vi "example test.vi"() -> ()   [LabVIEW 2013, in "Profibus Module tests.lvlib"]
uses:
  Profibus Module tests.lvlib
  <vilib>/Utility/RT CPU Load.ctl
  configuration/Profibus Module configuration.lvclass
  execution/Profibus Module runtime.lvclass
  <vilib>/NI/Tag Bus/tag/Data Type.ctl
  <vilib>/NI/Tag Bus Module Framework/channel/channel classification.ctl
  channel/Profibus channel.lvclass
  <vilib>/userdefined/High Color/nirio_resource_hc.ctl
  <vilib>/NI/Tag Bus Module Framework/FPGA manager/methods.ctl
  <vilib>/Platform/TimedLoop/XDataNode/timing_clust.ctl
  <vilib>/Platform/TimedLoop/XDataNode/nitl_modes.ctl
  <vilib>/Platform/TimedLoop/XDataNode/wakeup.ctl
  configuration/endianness setting.ctl
  configuration/slave diagnostic configuration.ctl
  <vilib>/NI/Tag Bus Module Framework/channel/TBM channel.lvclass
  configuration/error throw specification.ctl
  <vilib>/NI/Tag Bus Module Framework/channel/TBM channel.lvclass/TBM channel.ctl
  channel/Profibus channel.lvclass/Profibus channel.ctl
  <vilib>/NI/Tag Bus/tag/tag descriptor.lvclass/tag descriptor.ctl
  configuration/Profibus Module configuration.lvclass/Profibus Module configuration.ctl
  <vilib>/NI/Tag Bus/dictionary/data dictionary.lvclass/data dictionary.ctl
  <vilib>/NI/Tag Bus/dictionary/lookup polymorphs/locate Array of U8.vi
  <vilib>/NI/Tag Bus/table/data polymorphs/write one/write U16.vi
  <vilib>/NI/Tag Bus/table/data polymorphs/write one/write Array of U8.vi
  <vilib>/NI/Tag Bus/table/data polymorphs/read one/read Array of U8.vi
  <vilib>/NI/Tag Bus Module Framework/channel/Write channel classification.vi
  channel/Write slave.vi
  channel/Write byte.vi
  channel/Write bit.vi
  <vilib>/NI/Tag Bus/tag/write data type.vi
  <vilib>/NI/Tag Bus/tag/write tag name.vi
  configuration/Write byte orders.vi
  configuration/Write slave diagnostics.vi
  <vilib>/NI/Tag Bus/dictionary/search/find data index.vi
  <vilib>/NI/Tag Bus/dictionary/search/search string list.vi
  <vilib>/FPGAPlugInAG/cRIO-9074/niLvFpga_Open_cRIO-9074.vi
  <vilib>/rvi/interface/common/dynamic/niFpgaDynamicAddResources.vi
  <vilib>/FPGAPlugInAG/Dynamic/niLvFpga_Reset_Dynamic.vi
  <vilib>/FPGAPlugInAG/Dynamic/niLvFpga_Run_Dynamic.vi
  <vilib>/NI/Tag Bus/dictionary/tag not found.vi
  <vilib>/rvi/interface/common/niFpgaWaitOnOcc.vi
  <vilib>/Utility/error.llb/Error Cluster From Error Code.vi
  <vilib>/rvi/errors/niLvFpgaAdjustHostInterfaceError.vi
  <vilib>/FPGAPlugInAG/Dynamic/niLvFpga_Close_Dynamic.vi
  <vilib>/platform/TimedLoop/XDataNode/XDataNode.xnode
  <vilib>/rvi/interface/nirviOpenFPGA/nirviOpenFPGA.xnode
  FPGA Bitfiles/ProfibusModule_FPGA9074_FPGAMain_bIHCZjrjays.lvbitx
  execution/FPGA Main.vi
  <vilib>/rvi/interface/nirviMethod/nirviMethod.xnode
  <vilib>/rvi/interface/nirviCloseFPGA/nirviCloseFPGA.xnode
  <vilib>/NI/Tag Bus/dictionary/data dictionary.lvclass
  <vilib>/NI/Tag Bus/table/data table.lvlib
  <vilib>/NI/Tag Bus/tag/tag descriptor.lvclass
  <vilib>/NI/Configuration Framework/serializable configuration/NISE_CEF_serializable configuration.lvclass
  <vilib>/NI/Tag Bus Module Framework/FPGA manager/FPGA manager.lvlib
  <vilib>/NI_Real-Time Target Support.lvlib
  <vilib>/Platform/TimedLoop/XDataNode/XDNodeRunTimeDep.lvlib
  <vilib>/FPGAPlugInAG/Dynamic/niLvFpga_ReadFifo_Dynamic.vi
  <vilib>/rvi/errors/niLvFpgaMergeErrorWithErrorCode.vi
  <vilib>/ptbypt/NI_PtbyPt.lvlib
  <vilib>/NI/Tag Bus/dictionary/lookup polymorphs/locate U16.vi
panel:
  out "class name":string
  out "configuration out":refnum<class "Profibus Module configuration.lvclass">
  out "diag":u8[](array[numeric])
  out "value":u8[](array[numeric])
  in  "value 2":u16
  out "*(type *) &x 2":u64
  out "rio init error":errorcluster
  out "in mean":dbl
  out "out mean":dbl
  out "out":dbl
  out "in":dbl
  out "Elements Remaining":u32
  in  "millisecond multiple":u32=100
  out "CPU loads":T1[](array[typedef]) {"ISR (%)" format="%#.2f"; "Idle (%)" format="%#.2f"; "Background (%)" format="%#.2f"; "Normal (%)" format="%#.2f"; "Above Normal (%)" format="%#.2f"; "High (%)" format="%#.2g"; "Timed Structures (%)" format="%#.2g"; "Time Critical (%)" format="%#.2g"; "Total (%)" format="%#.2g"}
  in  "stop cpu":bool
  out "*(type *) &x":u64
  out "error out":errorcluster
  in  "stop":bool
  out "final error":errorcluster
  out "output error":errorcluster
  out "input error":errorcluster
  out "output lookup error":errorcluster
  out "input lookup error":errorcluster
  out "init error":errorcluster
  out "correct execution settings":bool
  out "serialization problem":errorcluster
  out "invalid configuration":errorcluster
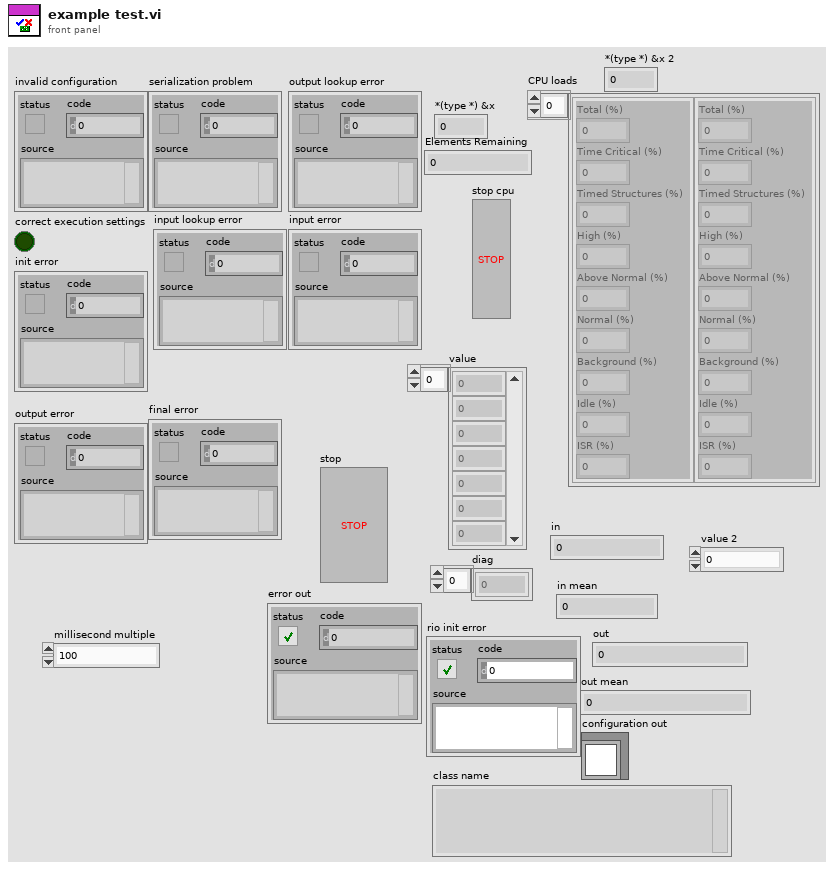
[diagram p1: front panel]
types:
  T1 = typedef "NI_Real-Time Target Support.lvlib/RT CPU Load.ctl" = cluster{"Total (%)":dbl, "Time Critical (%)":dbl, "Timed Structures (%)":dbl, "High (%)":dbl, "Above Normal (%)":dbl, "Normal (%)":dbl, "Background (%)":dbl, "Idle (%)":dbl, "ISR (%)":dbl}
  T2 = typedef "TBM channel.lvclass/channel classification.ctl" = enum16{"input data", "output data", "processing parameter", "processing result"}
  T3 = typedef "tag bus.lvlib/tag descriptor.lvclass/Data Type.ctl" = enum16{"Double", "Single", "I64", "I32", "I16", "I8", "U64", "U32", "U16", "U8", "Boolean", "String", "Array of Double", "Array of Single", "Array of I64", "Array of I32", "Array of I16", "Array of I8", "Array of U64", "Array of U32", "Array of U16", "Array of U8", "Array of Boolean", "Array of String"}
  T4 = typedef "Profibus Module configuration.lvclass/slave diagnostic configuration.ctl" = cluster{"slave":i8, "report":bool, "channel":refnum<class "TBM channel.lvclass">, "error specs":T5[]}
  T5 = typedef "Profibus Module configuration.lvclass/error throw specification.ctl" = cluster{"byte":i32, "bit":i32, "inverted?":bool, "error":i32}
  T6 = typedef "Profibus Module configuration.lvclass/endianness setting.ctl" = cluster{"slave":i8, "big endian":bool}
  T7 = typedef "nirio_resource_hc.ctl" = tag
  T8 = typedef "FPGA manager.lvlib/methods.ctl" = enum16{"initialize bitfile", "cache bitfile", "locate bitfile", "close bitfile", "clear manager"}
  T9 = typedef "TBM channel.lvclass/data tables.ctl" = cluster{"input data":T10, "processing parameter":T10, "processing result":T10, "output data":T10}
  T10 = typedef "tag bus.lvlib/dictionary table pair.ctl" = cluster{"data dictionary":refnum<class "data dictionary.lvclass">, "data table":T11}
  T11 = typedef "tag bus.lvlib/data table.lvlib/data table.ctl" = cluster{"Double":dbl[], "Single":sgl[], "I64":i64[], "I32":i32[], "I16":i16[], "I8":i8[], "U64":u64[], "U32":u32[], "U16":u16[], "U8":u8[], "Boolean":bool[], "String":string[], "Array of Double":cluster{"DBL Array":dbl[]}[], "Array of Single":cluster{"SGL Array":sgl[]}[], "Array of I64":cluster{"I64 Array":i64[]}[], "Array of I32":cluster{"I32 Array":i32[]}[], "Array of I16":cluster{"I16 Array":i16[]}[], "Array of I8":cluster{"I8 Array":i8[]}[], "Array of U64":cluster{"U64 Array":u64[]}[], "Array of U32":cluster{"U32 Array":u32[]}[], "Array of U16":cluster{"U16 Array":u16[]}[], "Array of U8":cluster{"U8 Array":u8[]}[], "Array of Boolean":cluster{"Boolean Array":bool[]}[], "Array of String":cluster{"String Array":string[]}[]}
  T12 = typedef "TBM module execution interface.lvclass/execution settings.ctl" = cluster{"reads inputs":bool, "processes data":bool, "writes outputs":bool}
  T13 = typedef "XDNodeRunTimeDep.lvlib/timing_clust.ctl" = cluster{"Expected End [f-1]":u64, "Actual End [f-1]":u64, "Finished Late? [f-1]":bool, "Expected End [i-1]":u64, "Actual End [i-1]":u64, "Finished Late? [i-1]":bool, "Expected Start [i]":u64, "Actual Start [i]":u64, "Expected Start [f]":u64, "Actual Start [f]":u64, "Source Name":string, "Structure Name":string, "Period":i64, "Deadline":i64, "Offset":i64, "Start":i64, "Priority":i32, "Timeout":i32, "Mode":T14, "Wakeup Reason":T15, "Error":errorcluster, "Source Type":string, "Secondary Source Type":string, "Global End Time":u64, "Global Start Time":u64, "Frame Duration":u64, "Iteration Duration":u64, "Assigned CPU":i32, "I/O Scan Engine Mode":u32}
  T14 = typedef "XDNodeRunTimeDep.lvlib/nitl_modes.ctl" = enum32{"No Change", "Process missed periods, maintain original phase", "Discard missed periods, maintain original phase", "Process missed periods, ignore original phase", "Discard missed periods, ignore original phase"}
  T15 = typedef "XDNodeRunTimeDep.lvlib/wakeup.ctl" = enum32{"Normal", "Aborted", "Asynchronous wakeup", "Timing source error", "Timed loop error", "Timeout"}
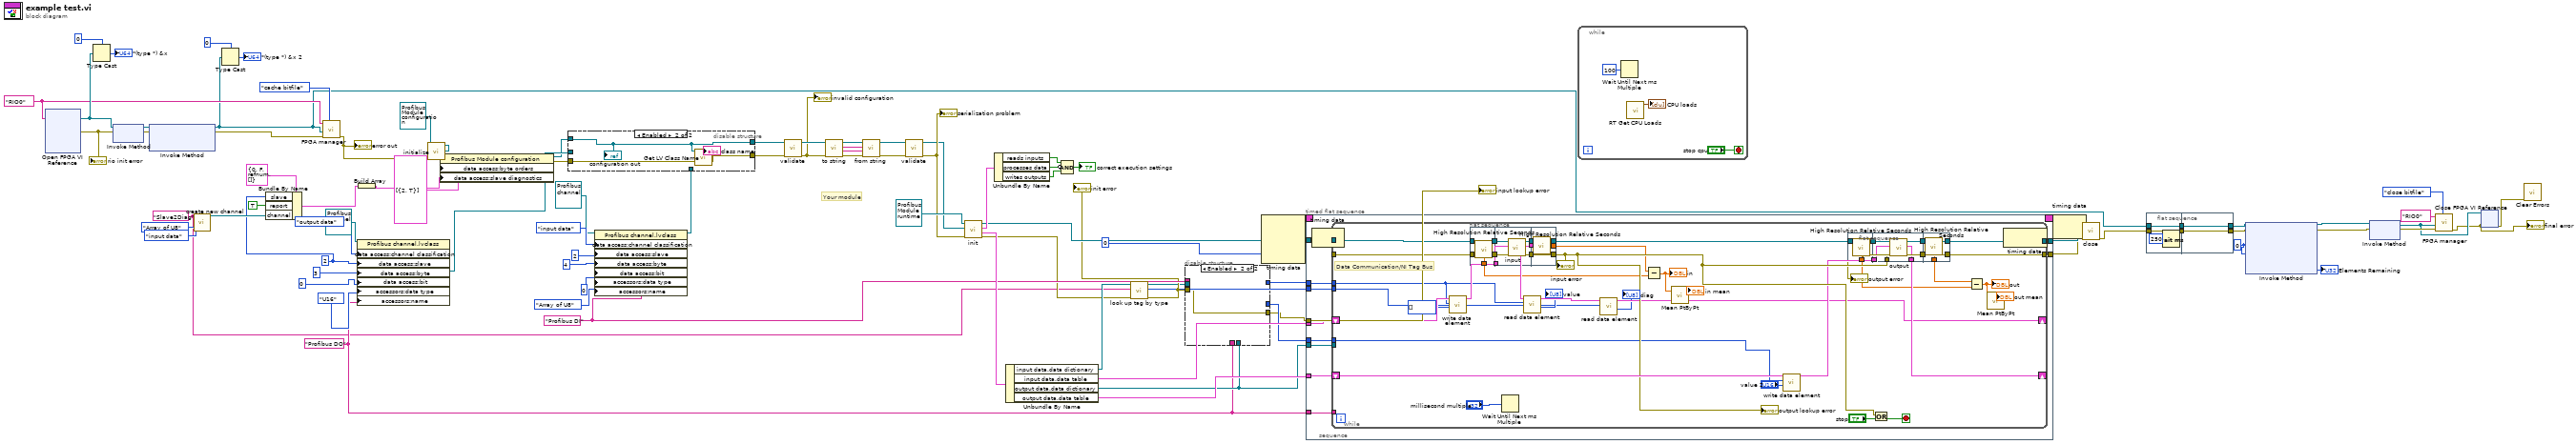
[diagram p0: block diagram]
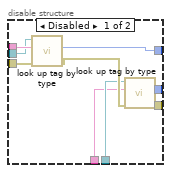
[diagram p2: hidden frame]
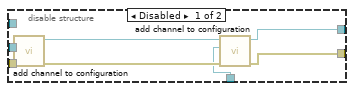
[diagram p3: hidden frame]
diagram:
  w4 = "Slave2Diag" ("channel name")
  w33 = u32 0 ("Number of Elements")
  w31 = T7 "RIO0" ("RIO resource")
  w54 = "Profibus DI" ("name")
  w11 = i8 2 ("slave")
  w18 = "Profibus DO" ("name")
  # "Your module"
  n1 = xnode "Open FPGA VI Reference"("resource name"=w31) -> ("FPGA VI Reference Out"=w45:refnum<k20>, "error out"=w53:errorcluster)  [unwired: 1 in]
  "rio init error" <- w53
  n2 = Type Cast(type=u64 0, x=w45) -> (*(type *) &x=→"*(type *) &x":u64)
  n3 = xnode "Invoke Method"("FPGA VI Reference In"=w45, "error in"=w53) -> ("FPGA VI Reference Out"=w51:refnum<k20>, "error out"=w52:errorcluster)
  n4 = xnode "Invoke Method"("FPGA VI Reference In"=w51, "error in"=w52) -> ("FPGA VI Reference Out"=w1:refnum<k20>, "error out"=w50:errorcluster)  [unwired: 1 in]
  n5 = call <vilib>:"create new channel.vi"("channel classification"=channel_classification."input data", "data type"=Data_Type."Array of U8", "channel name"=w4) -> ("channel"=w12:refnum<class "TBM channel.lvclass">)  [unwired: 8 in]
  n6 = Type Cast(type=u64 0, x=w1) -> (*(type *) &x=→"*(type *) &x 2":u64)
  n7 = Bundle By Name(cluster=T4 {"slave"=0, "report"=FALSE, "channel"=refnum, "error specs"=[]} ("diagnostics settings"), "slave"=w11, "report"=TRUE, "channel"=w12) -> (w15:T4)
  n8 = call <vilib>:"FPGA manager.vi"("action"=methods."cache bitfile", "error in"=w50, "bitfile to cache"=w1, "RIO resource"=w31) -> ("error out"=w48:errorcluster)  [unwired: 5 in, 2 out]
  "error out" <- w48
  n9 = property class="Profibus channel.lvclass"(reference=refnum<class "Profibus channel.lvclass"> refnum ("Profibus channel.lvclass"), "data access:channel classification"=channel_classification."output data" ("channel classification"), "data access:slave"=w11, "data access:byte"=3 ("DO byte"), "data access:bit"=0 ("DO bit"), "accessors:data type"=Data_Type."U16" ("data type"), "accessors:name"=w18) -> (reference out=w55:refnum<class "Profibus channel.lvclass">)  [unwired: 1 in, 1 out]
  n10 = Build Array(w15) -> (w14:T4[])
  n11 = call <vilib>:"initialize.vi"("error in"=w48, "configuration in"=refnum<class "Profibus Module configuration.lvclass"> refnum ("tag bus configurable plugin module configuration")) -> ("error out"=w68:errorcluster, "configuration out"=w23:refnum<class "Profibus Module configuration.lvclass">)  [unwired: 7 in, 1 out]
  n12 = property class="Profibus Module configuration"(reference=w23, error in=w68, "data access:byte orders"=T6[] [{"slave"=2, "big endian"=TRUE}] ("byte orders"), "data access:slave diagnostics"=w14) -> (reference out=w2:refnum<class "Profibus Module configuration.lvclass">, error out=w24:errorcluster)
  n13 = property class="Profibus channel.lvclass"(reference=refnum<class "Profibus channel.lvclass"> refnum ("Profibus channel.lvclass"), "data access:channel classification"=channel_classification."input data" ("channel classification"), "data access:slave"=i8 2 ("slave"), "data access:byte"=4 ("DI byte"), "data access:bit"=0 ("DI bit"), "accessors:data type"=Data_Type."Array of U8" ("data type"), "accessors:name"=w54) -> (reference out=w56:refnum<class "Profibus channel.lvclass">)  [unwired: 1 in, 1 out]
  n14 = disable-structure shown="Enabled" {
    disable-tunnel: [w101 w103] -> w71
    disable-tunnel: [w100 w104] -> w70
    disable-tunnel: w56 -> [w97 _]
    disable-tunnel: w55 -> [w96 _]
    disable-tunnel: w24 -> [w95 w104]
    disable-tunnel: w2 -> [_ w103]
    frame Disabled {
      n15 = call "add channel to configuration.vi"("error in"=w95, "TBM channel in"=w96) -> ("error out"=w98:errorcluster, "Profibus Module configuration out"=w99:refnum<class "Profibus Module configuration.lvclass">)  [unwired: 8 in]
      n16 = call "add channel to configuration.vi"("error in"=w98, "TBM channel in"=w97, "Profibus Module configuration in"=w99) -> ("error out"=w100:errorcluster, "Profibus Module configuration out"=w101:refnum<class "Profibus Module configuration.lvclass">)  [unwired: 7 in]
    }
    frame Enabled {
      n17 = call <vilib>:"Get LV Class Name.vi"("object"=w103) -> ("class name"=→"class name":string)  [unwired: 9 in, 1 out]
      "configuration out" <- w103
    }
  }
  n18 = call-dynamic "validate.vi"("error in"=w70, "Profibus Module configuration in"=w71) -> ("error out"=w93:errorcluster, "Profibus Module configuration out"=w94:refnum<class "Profibus Module configuration.lvclass">)  [unwired: 8 in]
  "invalid configuration" <- w93
  n19 = call-dynamic "to string.vi"("error in"=w93, "Profibus Module configuration in"=w94) -> ("error out"=w89:errorcluster, "data"=w90:string, "version"=w91:string, "Profibus Module configuration out"=w92:refnum<class "Profibus Module configuration.lvclass">)  [unwired: 6 in]
  n20 = call-dynamic "from string.vi"("error in"=w89, "data"=w90, "version"=w91, "Profibus Module configuration in"=w92) -> ("error out"=w87:errorcluster, "Profibus Module configuration out"=w88:refnum<class "Profibus Module configuration.lvclass">)  [unwired: 6 in]
  n21 = call-dynamic "validate.vi"("error in"=w87, "Profibus Module configuration in"=w88) -> ("error out"=w85:errorcluster, "Profibus Module configuration out"=w84:refnum<class "Profibus Module configuration.lvclass">)  [unwired: 8 in]
  "serialization problem" <- w85
  n22 = call-dynamic "init.vi"("error in"=w85, "TBM module configuration in"=w84, "Profibus Module runtime in"=refnum<class "Profibus Module runtime.lvclass"> refnum ("tag bus configurable plugin module")) -> ("error out"=w5:errorcluster, "data allocations"=w78:T9, "execution settings"=w83:T12, "Profibus Module runtime out"=w76:refnum<class "Profibus Module runtime.lvclass">)  [unwired: 5 in]
  n23 = Unbundle By Name(w83) -> ("reads inputs"=w80:bool, "processes data"=w82:bool, "writes outputs"=w81:bool)
  n24 = Unbundle By Name(w78) -> ("input data.data dictionary"=w7:refnum<class "data dictionary.lvclass">, "input data.data table"=w77:T11, "output data.data dictionary"=w20:refnum<class "data dictionary.lvclass">, "output data.data table"=w74:T11)
  n25 = Compound Arithmetic op=AND(w80, invert w82, w81) -> (→"correct execution settings":bool)
  n26 = call-poly <vilib>:"look up tag by type.vi"("error in"=w5, "name"=w4, "data dictionary in"=w7) -> ("error out"=w8:errorcluster, "index"=w3:i32, "data dictionary out"=w6:refnum<class "data dictionary.lvclass">)  [unwired: 6 in]
  "init error" <- w8
  n27 = disable-structure shown="Enabled" {
    disable-tunnel: [w113 _] -> w75
    disable-tunnel: w54 -> [w112 _]
    disable-tunnel: w20 -> [w110 _]
    disable-tunnel: [w109 _] -> w19
    disable-tunnel: w18 -> [w108 _]
    disable-tunnel: [w107 w114] -> w17
    disable-tunnel: w8 -> [w106 w114]
    disable-tunnel: w6 -> [w105 _]
    frame Disabled {
      n28 = call-poly <vilib>:"look up tag by type.vi"("error in"=w106, "name"=w112, "data dictionary in"=w105) -> ("error out"=w111:errorcluster, "index"=w113:i32)  [unwired: 6 in, 1 out]
      n29 = call-poly <vilib>:"look up tag by type.vi"("error in"=w111, "name"=w108, "data dictionary in"=w110) -> ("error out"=w107:errorcluster, "index"=w109:i32)  [unwired: 6 in, 1 out]
    }
    frame Enabled {
    }
  }
  "input lookup error" <- w17
  n30 = node-c288(0 ("Processor")) -> (w42:T13)  [unwired: 3 in]
  n31 = timed-sequence {
    timing: w42 -> [_]
    timing-out: [_] -> w41
    tunnel: w77 -> [w125]
    tunnel: w76 -> [w124]
    tunnel: w17 -> [w123]
    tunnel: w75 -> [w122]
    tunnel: w20 -> [w121]
    tunnel: w74 -> [w120]
    tunnel: [w119] -> w73
    tunnel: [w118] -> w72
    tunnel: w18 -> [w117]
    tunnel: w19 -> [w116]
    tunnel: w3 -> [w115]
    n32 = timed-flat-sequence {
      tunnel: w125 -> [w136]
      tunnel: w124 -> [w135]
      tunnel: w123 -> [w134]
      tunnel: w122 -> [w133]
      tunnel: w121 -> [w132]
      tunnel: w120 -> [w131]
      tunnel: [w130] -> w119
      tunnel: [w129] -> w118
      tunnel: w117 -> [w128]
      tunnel: w116 -> [w127]
      tunnel: w115 -> [w126]
      n33 = node-c288() -> ()  [unwired: 1 in, 1 out]
      n34 = while {
        tunnel: w135 -> [w175]
        tunnel: w134 -> [w174]
        tunnel: w133 -> [w171]
        tunnel: w132 -> [_]
        tunnel: [w166] -> w130
        tunnel: [w161] -> w129
        shift-right: [w165] -> _
        shift-left: w131 -> [w170]
        shift-right: [w139] -> _
        shift-left: w136 -> [w176]
        tunnel: w128 -> [_]
        tunnel: w127 -> [w143]
        tunnel: w126 -> [w138]
        stop <- w144 stop-if-true
        # "Data Communication/NI Tag Bus"
        n35 = call-poly <vilib>:"write data element.vi"("value"=u8[] [], "index"=w171, "data table in"=w176) -> ("data table out"=w173:T11)  [unwired: 8 in]
        n36 = flat-sequence {
          tunnel: w174 -> [w189]
          tunnel: w175 -> [w190]
          tunnel: [w190] -> w157
          tunnel: [w189] -> w156
          tunnel: [w188] -> w151
          tunnel: w173 -> [w194]
          tunnel: [w193] -> w160
          tunnel: [w192] -> w159
          tunnel: [w191] -> w158
          tunnel: w157 -> [w196]
          tunnel: w156 -> [w195]
          tunnel: [w198] -> w168
          tunnel: [w199] -> w169
          tunnel: [w200] -> w172
          tunnel: w160 -> [w200]
          tunnel: w159 -> [w199]
          tunnel: w158 -> [w198]
          tunnel: [w197] -> w152
          frame #0 {
            n37 = call <vilib>:"High Resolution Relative Seconds.vi"() -> ("relative seconds"=w188:dbl)
          }
          frame #1 {
            n38 = call-dynamic "input.vi"("error in"=w195, "data table in"=w194, "Profibus Module runtime in"=w196) -> ("error out"=w192:errorcluster, "data table out"=w193:T11, "Profibus Module runtime out"=w191:refnum<class "Profibus Module runtime.lvclass">)  [unwired: 6 in]
          }
          frame #2 {
            n39 = call <vilib>:"High Resolution Relative Seconds.vi"() -> ("relative seconds"=w197:dbl)
          }
        }
        n40 = Wait Until Next ms Multiple(millisecond multiple="millisecond multiple") -> ()  [unwired: 1 out]
        n41 = call-poly <vilib>:"read data element.vi"("index"=w171, "data table in"=w172) -> ("value"=→"value":u8[], "data table out"=w164:T11)  [unwired: 8 in]
        n42 = call-poly <vilib>:"read data element.vi"("index"=w138, "data table in"=w164) -> ("value"=→"diag":u8[], "data table out"=w139:T11)  [unwired: 8 in]
        n43 = Subtract(x=w152, y=w151) -> (x-y=w148:dbl)
        "in" <- w148
        n44 = call <vilib>:"Mean PtByPt.vi"("x"=w148) -> ("mean"=→"in mean":dbl)  [unwired: 3 in, 1 out]
        n45 = call-poly <vilib>:"write data element.vi"("value"="value 2", "index"=w143, "data table in"=w170) -> ("data table out"=w167:T11)  [unwired: 8 in]
        n46 = flat-sequence {
          tunnel: w168 -> [w178]
          tunnel: [w178] -> w155
          tunnel: [w177] -> w149
          tunnel: w169 -> [w184]
          tunnel: w167 -> [w182]
          tunnel: [w180] -> w165
          tunnel: w155 -> [w183]
          tunnel: [w181] -> w154
          tunnel: [w179] -> w153
          tunnel: [w186] -> w161
          tunnel: [w187] -> w166
          tunnel: w154 -> [w187]
          tunnel: w153 -> [w186]
          tunnel: [w185] -> w150
          frame #0 {
            n47 = call <vilib>:"High Resolution Relative Seconds.vi"() -> ("relative seconds"=w177:dbl)
          }
          frame #1 {
            n48 = call-dynamic "output.vi"("error in"=w184, "data table in"=w182, "Profibus Module runtime in"=w183) -> ("error out"=w179:errorcluster, "data table out"=w180:T11, "Profibus Module runtime out"=w181:refnum<class "Profibus Module runtime.lvclass">)  [unwired: 6 in]
          }
          frame #2 {
            n49 = call <vilib>:"High Resolution Relative Seconds.vi"() -> ("relative seconds"=w185:dbl)
          }
        }
        n50 = Or(x=w169, y="stop") -> (x .or. y?=w144:bool)
        n51 = Subtract(x=w150, y=w149) -> (x-y=w146:dbl)
        "out" <- w146
        n52 = call <vilib>:"Mean PtByPt.vi"("x"=w146) -> ("mean"=→"out mean":dbl)  [unwired: 3 in, 1 out]
        "output lookup error" <- w169
        "input error" <- w169
        "output error" <- w161
      }
      n53 = node-c288() -> ()  [unwired: 1 in, 1 out]
    }
  }
  n54 = while {
    stop <- "stop cpu" stop-if-true
    n55 = Wait Until Next ms Multiple(millisecond multiple=u32 100) -> ()  [unwired: 1 out]
    n56 = call <vilib>:"RT Get CPU Loads.vi"() -> ("CPU loads"=→"CPU loads":T1[])  [unwired: 10 in, 1 out]
  }
  n57 = node-c288(w41) -> ()  [unwired: 1 out]
  n58 = call-dynamic "close.vi"("error in"=w72, "Profibus Module runtime in"=w73) -> ("error out"=w39:errorcluster)  [unwired: 9 in]
  n59 = flat-sequence {
    tunnel: w1 -> [w207]
    tunnel: w39 -> [w208]
    tunnel: [w208] -> w30
    tunnel: [w207] -> w29
    tunnel: [w210] -> w38
    tunnel: [w209] -> w35
    tunnel: w30 -> [w210]
    tunnel: w29 -> [w209]
    frame #0 {
      n60 = Wait (ms)(milliseconds to wait=u32 250) -> ()  [unwired: 1 out]
    }
    frame #1 {
    }
  }
  n61 = xnode "Invoke Method"("FPGA VI Reference In"=w35, "error in"=w38, "Number of Elements"=w33, "Timeout (ms)"=w33) -> ("FPGA VI Reference Out"=w34:refnum<k20>, "error out"=w36:errorcluster, "Elements Remaining"=→"Elements Remaining":u32)  [unwired: 1 out]
  n62 = xnode "Invoke Method"("FPGA VI Reference In"=w34, "error in"=w36) -> ("FPGA VI Reference Out"=w28:refnum<k20>, "error out"=w37:errorcluster)
  n63 = call <vilib>:"FPGA manager.vi"("action"=methods."close bitfile", "error in"=w37, "bitfile to cache"=w28, "RIO resource"=T7 "RIO0") -> ("error out"=w27:errorcluster)  [unwired: 5 in, 2 out]
  "final error" <- w27
  n64 = xnode "Close FPGA VI Reference"("FPGA VI Reference In"=w28, "error in"=w27) -> ("error out"=w26:errorcluster)
  n65 = call <vilib>:"Clear Errors.vi"("error in (no error)"=w26) -> ()  [unwired: 6 in, 1 out]
